vi "MonitorHumedadTemperatura.vi"() -> ()   [LabVIEW 2025]
uses:
  <vilib>/Utility/error.llb/Trim Whitespace One-Sided.vi
panel:
  out "Húmedad %":dbl
  out "Gráfica húmedad":dbl(graph)
  in  "stop":bool
  out "Gráfica Temperatura":dbl(graph)
  out "Temperatura °C":dbl
  in  "Puerto":u16=5000
  in  "Dirección IP":string="192.168.4.1"
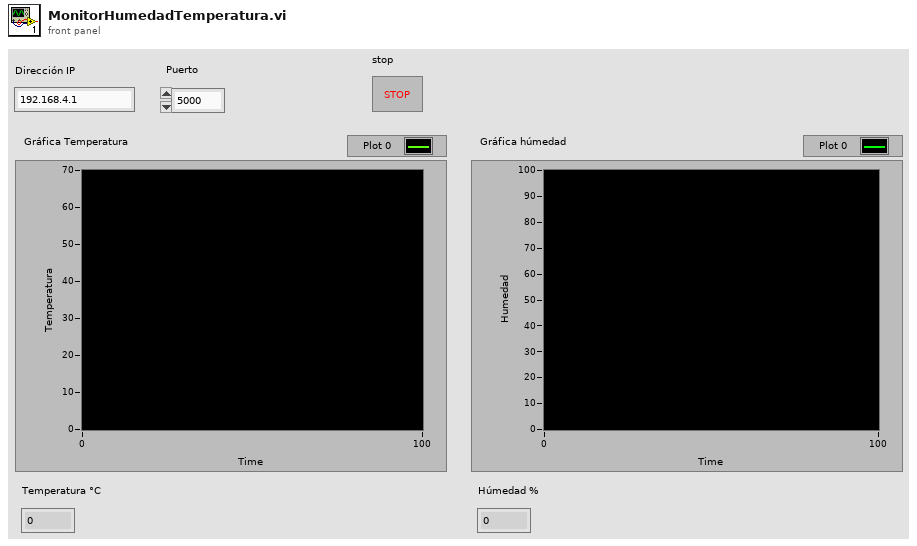
[diagram p1: front panel]
types:
  T1 = enum16{"Standard", "Buffered", "CRLF", "Immediate"}
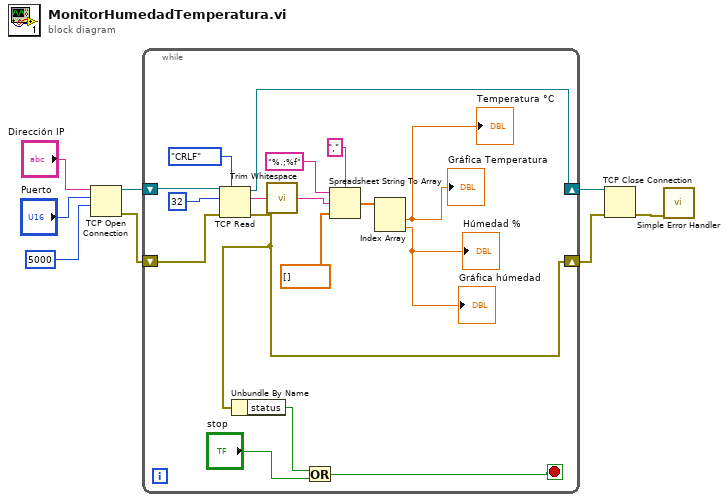
[diagram p0: block diagram]
diagram:
  n1 = TCP Open Connection(address="Dirección IP", remote port or service name="Puerto", timeout ms (60000)=5000) -> (connection ID=w8:refnum<k5>, error out=w7:errorcluster)  [unwired: 2 in]
  n2 = while {
    shift-right: [w21] -> w6
    shift-left: w7 -> [w23]
    shift-right: [w22] -> w5
    shift-left: w8 -> [w25]
    stop <- w17 stop-if-true
    n3 = TCP Read(connection ID=w25, bytes to read=32, error in (no error)=w23, 7:T1."CRLF" ("mode (standard)")) -> (connection ID out=w22:refnum<k5>, data out=w16:string, error out=w21:errorcluster)  [unwired: 1 in]
    n4 = Unbundle By Name(w21) -> ("status"=w20:bool)
    n5 = call <vilib>:"Trim Whitespace.vi"("string"=w16) -> ("trimmed string"=w12:string)  [unwired: 1 in]
    n6 = Or(x=w20, y="stop") -> (x .or. y?=w17:bool)
    n7 = Spreadsheet String To Array(delimiter (Tab)=",", format string="%.;%f", spreadsheet string=w12, array type (2D Dbl)=dbl[] []) -> (array=w11:dbl[])
    n8 = Index Array(array=w11) -> (element #1=→"Temperatura °C" →"Gráfica Temperatura":dbl, element #2=→"Gráfica húmedad" →"Húmedad %":dbl)  [unwired: 2 in]
  }
  n9 = TCP Close Connection(connection ID=w5, error in (no error)=w6) -> (error out=w1:errorcluster)  [unwired: 1 in, 1 out]
  n10 = call <vilib>:"Simple Error Handler.vi"("error in (no error)"=w1) -> ()  [unwired: 4 in, 5 out]
